vi "Open Template.vi"(8 "error in":errorcluster, 10 "Template":path, 11 "ILabVIEWFile in":refnum<class "Type Definition.lvclass">) -> (0 "error out":errorcluster, 3 "ILabVIEWFile out":refnum<class "Type Definition.lvclass">)   [LabVIEW 2026, in "Type Definition.lvclass"]
doc: "Open template (specified by file) and store reference in the class private data."
uses:
  Type Definition.lvclass
  C:/Users/juanj/Documents/hasbun_wood_engineering/github/py2vi/labview/Classes/LabVIEW File/LabVIEW File.lvclass
  <vilib>/Utility/traverseref.llb/TRef TravTarget.ctl
  LabVIEW File/LabVIEW File.lvclass/LabVIEW File.ctl
  Type Definition.lvclass/Type Definition.ctl
  LabVIEW File/Read VI Reference.vi
  LabVIEW File/LabVIEW File.lvclass
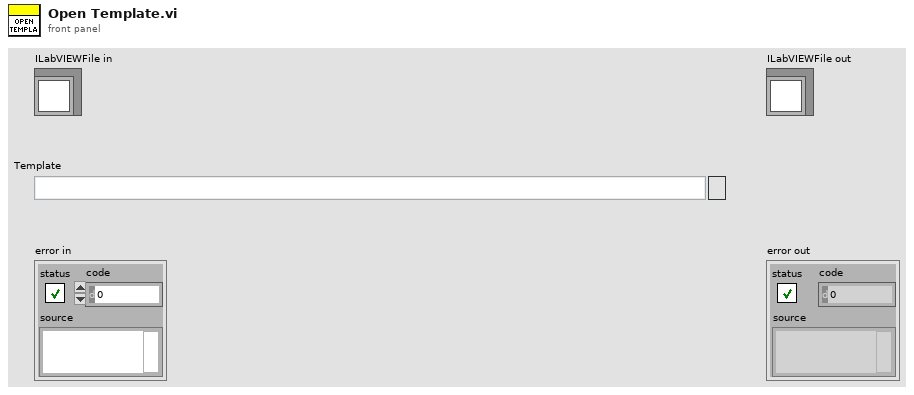
[diagram p1: front panel]
types:
  T1 = typedef "TRef TravTarget.ctl" = enum16{"FP", "BD", "Other"}
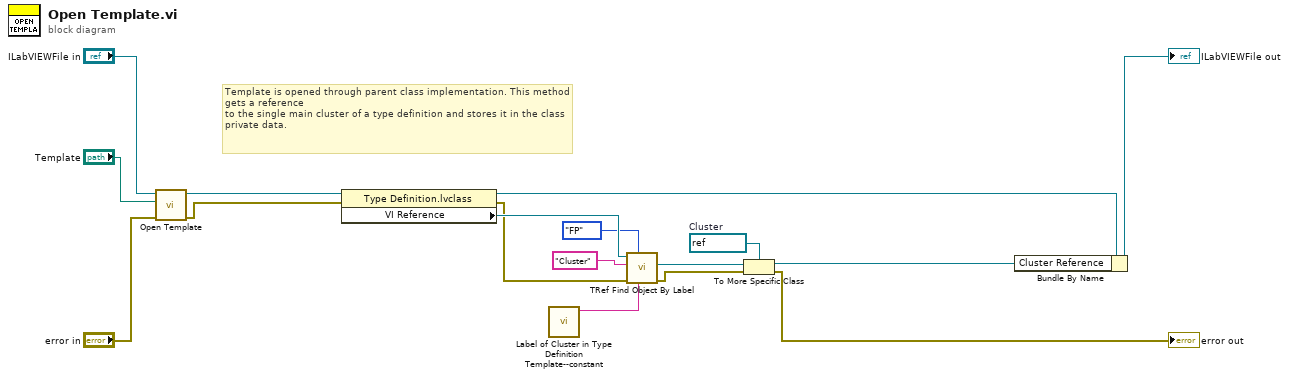
[diagram p0: block diagram]
diagram:
  w14 = refnum<vi> refnum  # Cluster
  # "Template is opened through parent class implementation. This method gets a reference\nto the single main cluster of a type definition and stores it in the class private data."
  n1 = call-parent "Open Template.vi"("error in"="error in", "Template"="Template", "ILabVIEWFile in"="ILabVIEWFile in") -> ("error out"=w15:errorcluster, "ILabVIEWFile out"=w10:refnum<class "Type Definition.lvclass">)  [unwired: 7 in]
  n2 = property class="Type Definition.lvclass"(reference=w10, error in=w15) -> (reference out=w8:refnum<class "Type Definition.lvclass">, error out=w5:errorcluster, "VI Reference"=w7:refnum<vi>)
  n3 = call "Label of Cluster in Type Definition Template--constant.vi"() -> ("Label of Cluster in Type Definition Template"=w4:string)  [unwired: 11 in]
  n4 = call <vilib>:"TRef Find Object By Label.vi"("Label"=w4, "Traverse Target"=TRef_TravTarget."FP", "error in (no error)"=w5, "Class Name"="Cluster", "VI Ref"=w7) -> ("error out"=w1:errorcluster, "Found Obj Ref"=w2:refnum<vi>)  [unwired: 3 in, 2 out]
  n5 = To More Specific Class(target class=w14, reference=w2, error in=w1) -> (specific class reference=w12:refnum<vi>, error out=→"error out":errorcluster)
  n6 = Bundle By Name(cluster=w8, "Cluster Reference"=w12) -> (→"ILabVIEWFile out":refnum<class "Type Definition.lvclass">)
